vi "PowerSpectrum.vi"(8 "error in (no error)":errorcluster, 9 "averaging parameters":T1={"averaging mode"=enum."No averaging", "weighting mode"=enum."Exponential", "number of averages"=10, "linear mode"=enum."One shot"}, 10 "Window":string, 11 "Data In":waveform(dbl)) -> (0 "error out":errorcluster, 3 "Array of Waveforms":waveform(dbl)[](array[waveform]), 5 "power spectrum [dB EU]":cluster{"f0":dbl, "df":dbl, "magnitude":dbl[]})   [LabVIEW 2026, in "Calculations.lvlib"]
uses:
  Calculations.lvlib
  <vilib>/addons/Sound and Vibration/svt_Integration/SVPO Integration (1 CH DBL WDT).vi
  <vilib>/Analysis/5stat.llb/RMS (DBL).vi
  <vilib>/addons/_NISVFA/_Baseband FFT/subVIs/svfa_Convert to One-Sided Power Spectrum.vi
  <vilib>/Analysis/2dsp.llb/Power Spectrum.vi
  <vilib>/Analysis/2dsp.llb/Power Spectrum (DBL).vi
  <vilib>/addons/_NISVFA/_Shared subVIs/Windowing/svfa_Scaled Time Domain Window (Array).vi
  <vilib>/addons/_NISVFA/_Spectrum Processing/SVFA Get Spectrum Subset.vi
  <vilib>/addons/_NISVFA/_Spectrum Processing/SVFA Get Spectrum Subset (1 Ch).vi
  <vilib>/addons/_NISVFA/_Shared subVIs/Common/svc_Window Parameters.vi
  <vilib>/addons/_NISVFA/_Shared subVIs/Common/svc_Spectrum Units.vi
  <vilib>/addons/_NISVFA/_Spectrum Processing/SVFA Unit Conversion.vi
  <vilib>/addons/_NISVFA/_Spectrum Processing/SVFA Unit Conversion (1 Ch).vi
  <vilib>/addons/_NISVFA/_Spectrum Processing/subVIs/svfa_Spectrum Info Window to windowTd Type Def.vi
  <vilib>/addons/Sound and Vibration/svt_Integration/SVPO Integration (1 CH DBL WDT) with IC.vi
  <vilib>/Analysis/4window.llb/Force Window.vi
  <vilib>/Analysis/4window.llb/Force Window (DBL).vi
  <vilib>/Analysis/4window.llb/Exponential Window.vi
  <vilib>/Analysis/4window.llb/Exponential Window (DBL).vi
  <vilib>/addons/_NISVFA/_Shared subVIs/Common/svc_Build Unit Label for Frequency Range.vi
  <vilib>/addons/_NISVFA/_Shared subVIs/Common/svc_Check Frequency Range in Spectrum.vi
  <vilib>/addons/_NISVFA/_Shared subVIs/Common/svc_Format Value (DBL).vi
  <vilib>/addons/_NISVFA/_Shared subVIs/Common/svc_Get Weighting Enum and Labels.vi
  <vilib>/addons/_NISVFA/_Shared subVIs/Common/svc_Engineering Units to Unit Label.vi
  <vilib>/addons/_NISVFA/_Shared subVIs/Common/svc_Surround NonAlpha String with Parentheses.vi
  <vilib>/dlg_ctls.llb/Space Constant.vi
  <vilib>/addons/_NISVFA/_Spectrum Processing/subVIs/svfa_Conversion Utility (spectrum info).vi
  <vilib>/addons/Sound and Vibration/svt_Integration/SVPO Integration (1 CH DBL Array) with IC.vi
  <vilib>/addons/_NISVFA/_Shared subVIs/Common/svc_Check Frequency Range in Bandwidth.vi
  <vilib>/addons/_NISVFA/_Shared subVIs/Common/svc_Convert Start and Stop to Start Index and Length.vi
  <vilib>/addons/_NISVFA/_Shared subVIs/Common/svc_Unit Label Lexical Class.vi
  <vilib>/addons/_NISVFA/_Spectrum Processing/subVIs/svfa_Peak to RMS to Peak2Peak.vi
  <vilib>/addons/_NISVFA/_Spectrum Processing/subVIs/svfa_Mag to Mag2.vi
  <vilib>/addons/_NISVFA/_Spectrum Processing/subVIs/svfa_Linear to dB.vi
  <vilib>/addons/_NISVFA/_Spectrum Processing/subVIs/svfa_dBrefA to dBrefB.vi
  <vilib>/addons/_NISVFA/_Spectrum Processing/subVIs/svfa_Spectrum to Spectral Density.vi
  <vilib>/Analysis/0measdsp.llb/Scaled Time Domain Window.vi
  <vilib>/Analysis/0measdsp.llb/Scaled Time Domain Window (DBL).vi
  <vilib>/Utility/error.llb/Error Cluster From Error Code.vi
  <vilib>/addons/_NISVFA/_Shared subVIs/Common/svc_Caller VI Returned in Error Source.vi
  <vilib>/addons/_NISVFA/_Shared subVIs/Common/svc_Convert Frequency to Frequency String.vi
  <vilib>/Analysis/4window.llb/window parameters.vi
  <vilib>/Analysis/4window.llb/Window Properties.vi
  <vilib>/Analysis/4window.llb/Window Properties by Name.vi
  <vilib>/addons/Sound and Vibration/svt_Integration/subVIs/svl_RC Filter Coefficients.vi
  <vilib>/addons/Sound and Vibration/svt_Integration/subVIs/svl_Design HighPass Filter.vi
  <vilib>/addons/Sound and Vibration/svt_Integration/subVIs/svl_Low Pass [Order 1] No State.vi
  <vilib>/addons/Sound and Vibration/svt_Integration/subVIs/svl_Apply Highpass Filter with IC.vi
  <vilib>/addons/Sound and Vibration/svt_Integration/subVIs/svl_Integration Units.vi
  <vilib>/addons/Sound and Vibration/svt_Level/SoundVib_VibrationLevel.lvlib
  <vilib>/gmath/NI_Gmath.lvlib
  <vilib>/Analysis/NI_AALPro.lvlib
  <vilib>/addons/Sound and Vibration/svt_Integration/SoundVib_Integration.lvlib
panel:
  in  "window":u32(ring)=1 items=["None", "Hanning", "Hamming", "Blackman-Harris", "Exact Blackman", "Blackman", "Flat Top", "4 Term B-Harris ", "7 Term B-Harris", "Low Sidelobe", "Force", "Exponential", "Blackman Nuttall", "Triangle", "Bartlett-Hanning", "Bohman", "Parzen", "Welch", "Kaiser", "Dolph-Chebyshev", "Gaussian"]
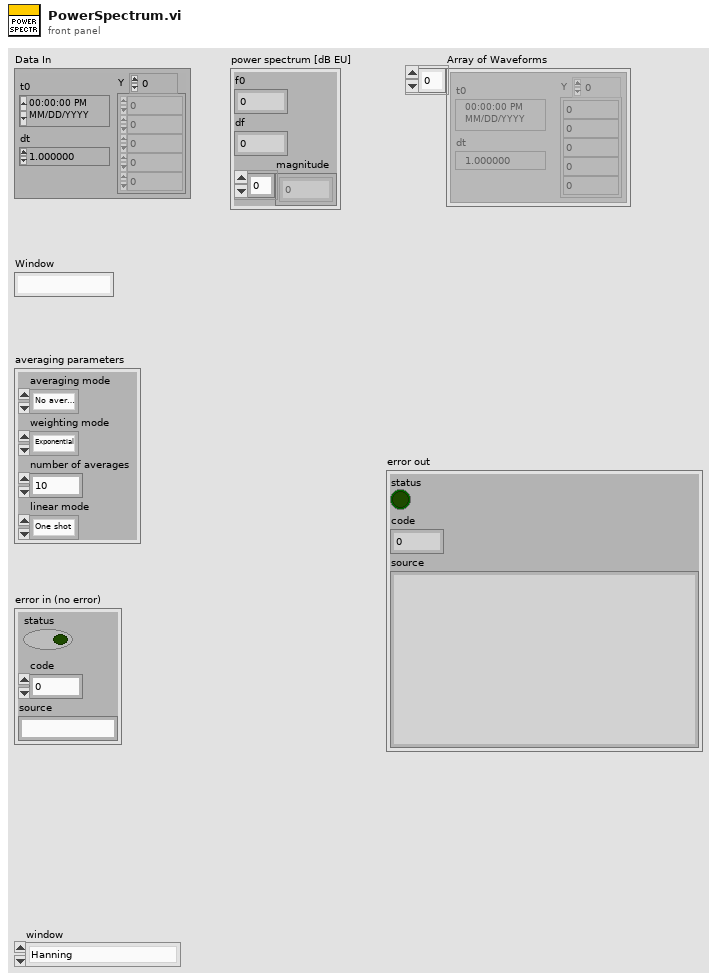
[diagram p1: front panel]
types:
  T1 = cluster{"averaging mode":enum16{"No averaging", "Vector averaging", "RMS averaging", "Peak hold"}, "weighting mode":enum16{"Linear", "Exponential"}, "number of averages":u32, "linear mode":enum16{"One shot", "Auto restart"}}
  T2 = typedef "svc_Spectrum Info.ctl" = cluster{"channel name":string, "description":string, "x-axis units":T3, "spectral info":cluster{"spectrum type":T4, "linear/dB":enum16{"linear", "dB"}, "window":u16, "window size":i32, "FFT size":i32}, "engineering units":T5, "custom label":string, "dB reference [EU]":dbl, "peak units":enum16{"rms", "peak", "peak-peak"}, "weighting filter":T6, "spectral density?":bool, "unit label":string, "spectrum skewed?":bool, "complimentary spectrum units":T7}
  T3 = typedef "svc_X-Axis Units.ctl" = u16
  T4 = typedef "svc_Spectrum Type.ctl" = enum16{"FFT Spectrum [complex]", "Amplitude [Magnitude]", "Power [Magnitude^2]", "Cross Spectrum [complex]", "Frequency Response [Complex]"}
  T5 = typedef "svc_Engineering Units Text Ring.ctl" = u16
  T6 = typedef "svc_Weighting Filter Text Ring.ctl" = u16
  T7 = typedef "svc_Complimentary Spectrum Units.ctl" = enum16{"none", "radians", "degrees", "cycles", "imaginary"}
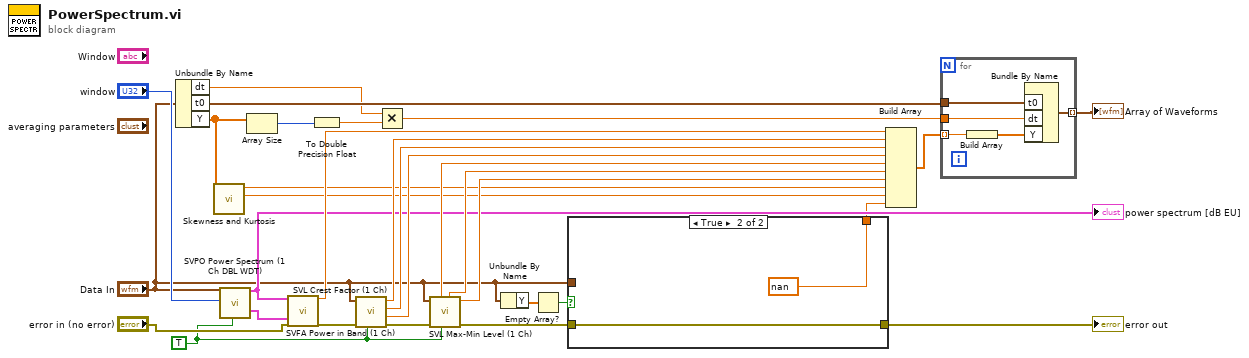
[diagram p0: block diagram]
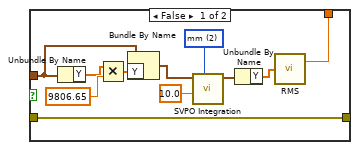
[diagram p2: hidden frame]
diagram:
  w8 = TRUE ("restart averaging")
  n1 = Unbundle By Name("Data In") -> ("dt"=w15:dbl, "t0"=w16:timestamp, "Y"=w10:dbl[])
  n2 = call <vilib>:"Skewness and Kurtosis.vi"("X"=w10) -> ("kurtosis"=w4:dbl, "skewness"=w5:dbl)  [unwired: 8 in, 1 out]
  n3 = call <vilib>:"SVPO Power Spectrum (1 Ch DBL WDT).vi"("scaled signal [EU]"="Data In", "window"="window", "restart averaging? (F)"=w8) -> ("power spectrum [EU^2 rms]"=w11:cluster{"f0":dbl, "df":dbl, "magnitude":dbl[]}, "spectrum info"=w20:T2)  [unwired: 14 in, 1 out]
  "power spectrum [dB EU]" <- w11
  n4 = Array Size(array=w10) -> (size(s)=w17:i32)
  n5 = call <vilib>:"SVFA Power in Band (1 Ch).vi"("spectrum"=w11, "spectrum info"=w20, "error in (no error)"="error in (no error)") -> ("power in band"=w21:dbl, "error out"=w22:errorcluster)  [unwired: 14 in, 1 out]
  n6 = To Double Precision Float(number=w17) -> (double precision float=w18:dbl)
  n7 = call <vilib>:"SVL Crest Factor (1 Ch).vi"("restart averaging (F)"=w8, "error in (no error)"=w22, "scaled signal [EU]"="Data In") -> ("error out"=w23:errorcluster, "RMS level [EU rms]"=w24:dbl, "peak level [EU]"=w25:dbl, "crest factor"=w26:dbl)  [unwired: 5 in]
  n8 = Multiply(x=w15, y=w18) -> (x*y=w19:dbl)
  n9 = call <vilib>:"SVL Max-Min Level (1 Ch).vi"("restart averaging (F)"=w8, "error in (no error)"=w23, "scaled signal [EU]"="Data In") -> ("error out"=w9:errorcluster, "max-min level [EU]"=w27:dbl, "min level [EU]"=w28:dbl, "max level [EU]"=w29:dbl)  [unwired: 4 in, 1 out]
  n10 = Unbundle By Name("Data In") -> ("Y"=w2:dbl[])
  n11 = Empty Array?(array=w2) -> (empty?=w1:bool)
  n12 = case shown="True" w1 {
    tunnel: w9 -> [w35 w43]
    tunnel: [w40 nan] -> w7
    tunnel: [w35 w43] -> w6
    tunnel: "Data In" -> [w33 _]
    frame False {
      w36 = 2 items=["no change"=-1, "m"=0, "mm"=2, "microns"=3, "in"=1, "mils"=5] ("length units")
      n13 = Unbundle By Name(w33) -> ("Y"=w34:dbl[])
      n14 = Multiply(x=w34, y=9806.65) -> (x*y=w32:dbl[])
      n15 = Bundle By Name(cluster=w33, "Y"=w32) -> (w31:waveform(dbl))
      n16 = call-poly <vilib>:"SVPO Integration.vi"("desired base units for length"=w36, "highpass cutoff frequency [Hz]"=10.0 ("highpass cutoff frequency  [Hz]"), "scaled signal [EU]"=w31) -> ("integrated signal [EU*s]"=w38:waveform(dbl))  [unwired: 8 in]
      n17 = Unbundle By Name(w38) -> ("Y"=w41:dbl[])
      n18 = call-poly <vilib>:"RMS.vi"("X"=w41) -> ("rms value"=w40:dbl)  [unwired: 1 out]
    }
    frame True {
    }
  }
  "error out" <- w6
  n19 = Build Array(w21, w26, w25, w24, w29, w28, w27, w5, w4, w7) -> (w30:dbl[])
  n20 = for {
    tunnel: w16 -> [w45]
    tunnel: w19 -> [w46]
    tunnel: w30 -> [w44] mode=indexing
    tunnel: [w48] -> w12 mode=indexing
    n21 = Build Array(w44) -> (w47:dbl[])
    n22 = Bundle By Name("t0"=w45, "dt"=w46, "Y"=w47) -> (w48:waveform(dbl))  [unwired: 1 in]
  }
  "Array of Waveforms" <- w12
